vi "GetTerminal.vi"(5 "UseGObject":bool, 6 "TerminalIndex":i32, 7 "Other Refnum":refnum<vi>, 8 "error in (no error)":errorcluster, 9 "TerminalType":string, 10 "Label":string, 11 "vi reference":refnum<vi>) -> (0 "error out":errorcluster, 1 "Terminal desc":string, 2 "Terminal out":refnum<vi>, 3 "dup VI Refnum":refnum<vi>)   [LabVIEW 2020]
uses:
  <vilib>/Utility/traverseref.llb/TRef TravTarget.ctl
  <vilib>/Utility/traverseref.llb/VI Scripting - Traverse.lvlib
panel:
  out "Array 2":string[](array[string])
  out "Array":string[](array[string])
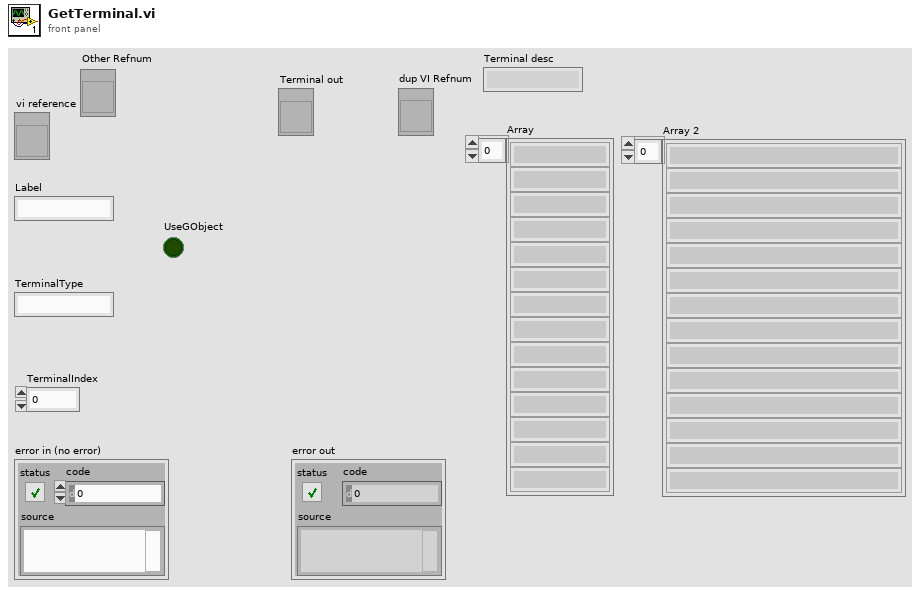
[diagram p1: front panel]
types:
  T1 = typedef "TRef TravTarget.ctl" = enum16{"FP", "BD", "Other"}
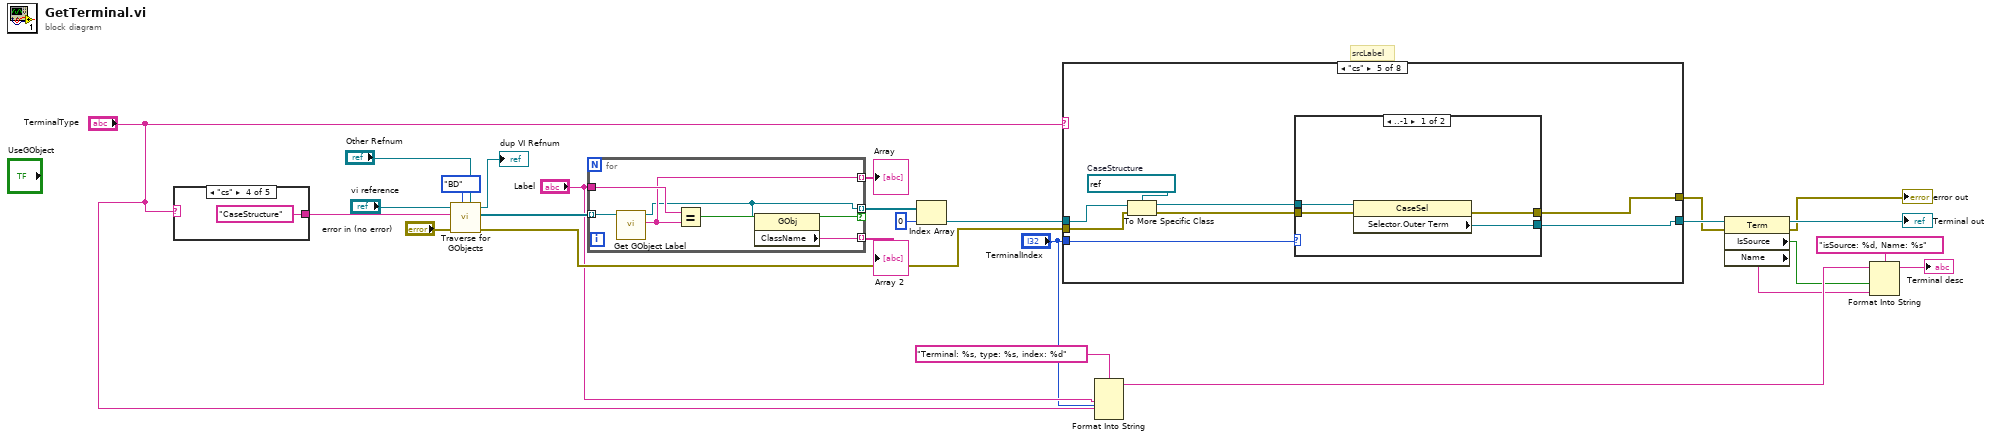
[diagram p0: block diagram]
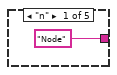
[diagram p2: hidden frame]
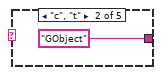
[diagram p3: hidden frame]
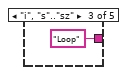
[diagram p4: hidden frame]
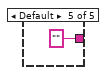
[diagram p5: hidden frame]
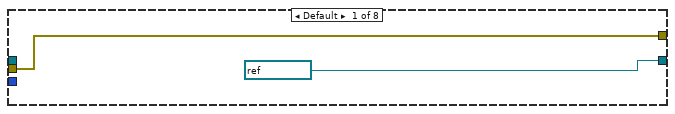
[diagram p6: hidden frame]
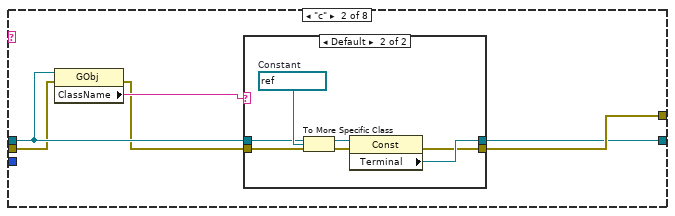
[diagram p7: hidden frame]
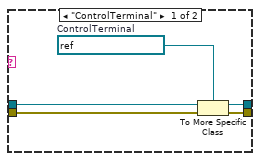
[diagram p8: hidden frame]
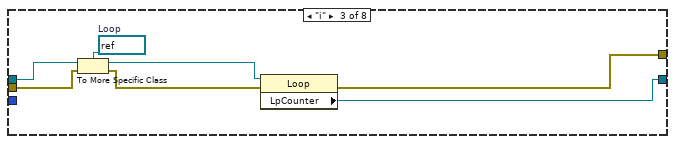
[diagram p9: hidden frame]
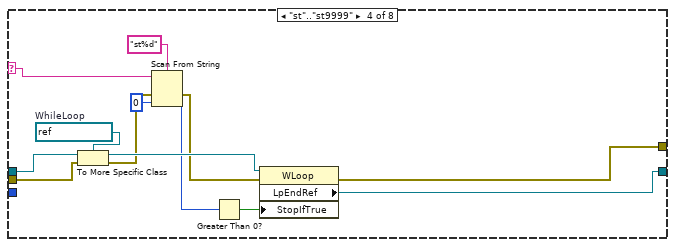
[diagram p10: hidden frame]
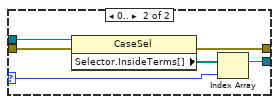
[diagram p11: hidden frame]
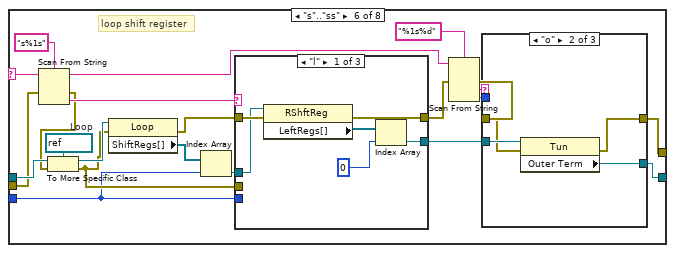
[diagram p12: hidden frame]
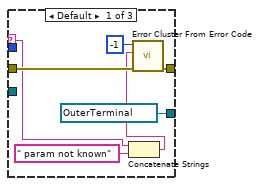
[diagram p13: hidden frame]
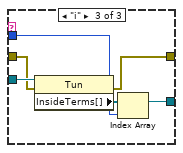
[diagram p14: hidden frame]
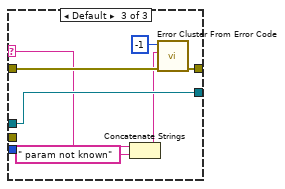
[diagram p16: hidden frame]
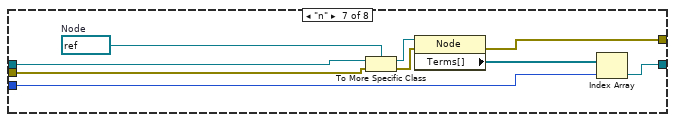
[diagram p17: hidden frame]
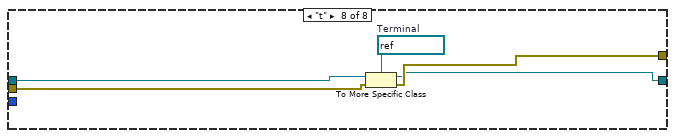
[diagram p18: hidden frame]
diagram:
  # "srcLabel"
  n1 = case shown="\"cs\"" "TerminalType" {
    tunnel: ["Node" "GObject" "Loop" "CaseStructure" ""] -> w25
    frame "n" {
    }
    frame "c", "t" {
    }
    frame "i", "s".."sz" {
    }
    frame "cs" {
    }
    frame Default {
    }
  }
  n2 = call <vilib>:"Traverse for GObjects.vi"("Other Refnum"="Other Refnum", "Traverse Target"=TRef_TravTarget."BD", "error in (no error)"="error in (no error)", "Class Name"=w25, "VI Refnum"="vi reference") -> ("error out"=w19:errorcluster, "References"=w26:refnum<vi>[], "dup VI Refnum"=→"dup VI Refnum":refnum<vi>)  [unwired: 3 in, 1 out]
  n3 = for {
    tunnel: w26 -> [w37] mode=indexing
    tunnel: "Label" -> [w35]
    tunnel: [w33] -> w23 mode=indexing if=w36
    tunnel: [w34] -> w17 mode=indexing
    tunnel: [w32] -> w16 mode=indexing
    n4 = call <vilib>:"Get GObject Label.vi"("GObject"=w37) -> ("Object Label"=w34:string, "dup GObject"=w33:refnum<vi>)  [unwired: 6 in, 3 out]
    n5 = Equal?(x=w35, y=w34) -> (x = y?=w36:bool)
    n6 = property class="GObj"(reference=w33) -> ("ClassName"=w32:string)  [unwired: 1 in, 2 out]
  }
  "Array" <- w17
  "Array 2" <- w16
  n7 = Index Array(array=w23, index=0) -> (element=w21:refnum<vi>)
  n8 = case shown="\"cs\"" "TerminalType" {
    selector: "TerminalType" -> [_ _ _ w70 _ w113 _ _]
    tunnel: w21 -> [_ w43 w64 w77 w85 w117 w158 w163]
    tunnel: [refnum<vi> refnum ("Terminal") w44 w63 w76 w79 w102 w155 w159] -> w13
    tunnel: "TerminalIndex" -> [_ _ _ _ w78 w109 w153 _]
    tunnel: w19 -> [w38 w42 w59 w72 w82 w105 w152 w161]
    tunnel: [w38 w45 w62 w75 w84 w98 w150 w160] -> w11
    frame Default {
    }
    frame "c" {
      n9 = property class="GObj"(reference=w43, error in=w42) -> (error out=w40:errorcluster, "ClassName"=w41:string)  [unwired: 1 out]
      n10 = case shown="Default" w41 {
        tunnel: [w49 w51] -> w45
        tunnel: [w48 w52] -> w44
        tunnel: w43 -> [w47 w56]
        tunnel: w40 -> [w46 w55]
        frame "ControlTerminal" {
          w50 = refnum<vi> refnum  # ControlTerminal
          n11 = To More Specific Class(target class=w50, reference=w47, error in=w46) -> (specific class reference=w48:refnum<vi>, error out=w49:errorcluster)
        }
        frame Default {
          w57 = refnum<vi> refnum  # Constant
          n12 = To More Specific Class(target class=w57, reference=w56, error in=w55) -> (specific class reference=w54:refnum<vi>, error out=w53:errorcluster)
          n13 = property class="Const"(reference=w54, error in=w53) -> (error out=w51:errorcluster, "Terminal"=w52:refnum<vi>)  [unwired: 1 out]
        }
      }
    }
    frame "i" {
      w61 = refnum<vi> refnum  # Loop
      n14 = To More Specific Class(target class=w61, reference=w64, error in=w59) -> (specific class reference=w60:refnum<vi>, error out=w58:errorcluster)
      n15 = property class="Loop"(reference=w60, error in=w58) -> (error out=w62:errorcluster, "LpCounter"=w63:refnum<vi>)  [unwired: 1 out]
    }
    frame "st".."st9999" {
      w74 = refnum<vi> refnum  # WhileLoop
      n16 = To More Specific Class(target class=w74, reference=w77, error in=w72) -> (specific class reference=w73:refnum<vi>, error out=w67:errorcluster)
      n17 = Scan From String(format string="st%d", input string=w70, error in=w67, default 1=0 ("default value 1")) -> (error out=w66:errorcluster, output 1=w69:i32)  [unwired: 1 in, 2 out]
      n18 = Greater Than 0?(x=w69) -> (x > 0?=w68:bool)
      n19 = property class="WLoop"(reference=w73, error in=w66, "StopIfTrue"=w68) -> (error out=w75:errorcluster, "LpEndRef"=w76:refnum<vi>)  [unwired: 1 out]
    }
    frame "cs" {
      w83 = refnum<vi> refnum  # CaseStructure
      n20 = To More Specific Class(target class=w83, reference=w85, error in=w82) -> (specific class reference=w81:refnum<vi>, error out=w80:errorcluster)
      n21 = case shown="..-1" w78 {
        selector: w78 -> [_ w90]
        tunnel: [w89 w95] -> w84
        tunnel: w81 -> [w88 w94]
        tunnel: w80 -> [w87 w93]
        tunnel: [w86 w91] -> w79
        frame ..-1 {
          n22 = property class="CaseSel"(reference=w88, error in=w87) -> (error out=w89:errorcluster, "Selector.Outer Term"=w86:refnum<vi>)  [unwired: 1 out]
        }
        frame 0.. {
          n23 = property class="CaseSel"(reference=w94, error in=w93) -> (error out=w95:errorcluster, "Selector.InsideTerms[]"=w92:refnum<vi>[])  [unwired: 1 out]
          n24 = Index Array(array=w92, index=w90) -> (element=w91:refnum<vi>)
        }
      }
    }
    frame "s".."ss" {
      w116 = refnum<vi> refnum  # Loop
      # "loop shift register"
      n25 = Scan From String(format string="s%1s", input string=w113, error in=w105) -> (remaining string=w96:string, error out=w104:errorcluster, output 1=w111:string)  [unwired: 2 in, 1 out]
      n26 = To More Specific Class(target class=w116, reference=w117, error in=w104) -> (specific class reference=w115:refnum<vi>, error out=w114:errorcluster)
      n27 = property class="Loop"(reference=w115, error in=w114) -> (error out=w110:errorcluster, "ShiftRegs[]"=w108:refnum<vi>[])  [unwired: 1 out]
      n28 = Index Array(array=w108, index=w109) -> (element=w107:refnum<vi>)
      n29 = case shown="\"l\"" w111 {
        selector: w111 -> [_ _ w145]
        tunnel: w114 -> [_ w141 _]
        tunnel: [w140 w141 w148] -> w103
        tunnel: w110 -> [w139 _ w147]
        tunnel: w109 -> [_ _ _]
        tunnel: [w138 w142 w149] -> w106
        tunnel: w107 -> [w137 w142 w149]
        frame "l" {
          n30 = property class="RShftReg"(reference=w137, error in=w139) -> (error out=w140:errorcluster, "LeftRegs[]"=w136:refnum<vi>[])  [unwired: 1 out]
          n31 = Index Array(array=w136, index=0) -> (element=w138:refnum<vi>)
        }
        frame "r" {
        }
        frame Default {
          n32 = Concatenate Strings(w145, " param not known" ("string")) -> (w144:string)
          n33 = call <vilib>:"Error Cluster From Error Code.vi"("error in (no error)"=w147, "error message (\"\")"=w144, "error code (0)"=-1) -> ("error out"=w148:errorcluster)  [unwired: 6 in]
        }
      }
      n34 = Scan From String(format string="%1s%d", input string=w96, error in=w103) -> (error out=w99:errorcluster, output 1=w100:string, output 2=w97:i32)  [unwired: 3 in, 2 out]
      n35 = case shown="\"o\"" w100 {
        selector: w100 -> [w121 _ _]
        tunnel: w106 -> [_ w128 w134]
        tunnel: [refnum<vi> refnum ("Outer Term") w127 w132] -> w102
        tunnel: w99 -> [w124 w126 w130]
        tunnel: [w123 w125 w129] -> w98
        tunnel: w97 -> [_ _ w131]
        frame Default {
          n36 = Concatenate Strings(w121, " param not known" ("string")) -> (w120:string)
          n37 = call <vilib>:"Error Cluster From Error Code.vi"("error in (no error)"=w124, "error message (\"\")"=w120, "error code (0)"=-1) -> ("error out"=w123:errorcluster)  [unwired: 6 in]
        }
        frame "o" {
          n38 = property class="Tun"(reference=w128, error in=w126) -> (error out=w125:errorcluster, "Outer Term"=w127:refnum<vi>)  [unwired: 1 out]
        }
        frame "i" {
          n39 = property class="Tun"(reference=w134, error in=w130) -> (error out=w129:errorcluster, "InsideTerms[]"=w133:refnum<vi>[])  [unwired: 1 out]
          n40 = Index Array(array=w133, index=w131) -> (element=w132:refnum<vi>)
        }
      }
    }
    frame "n" {
      w157 = refnum<vi> refnum  # Node
      n41 = To More Specific Class(target class=w157, reference=w158, error in=w152) -> (specific class reference=w156:refnum<vi>, error out=w151:errorcluster)
      n42 = property class="Node"(reference=w156, error in=w151) -> (error out=w150:errorcluster, "Terms[]"=w154:refnum<vi>[])  [unwired: 1 out]
      n43 = Index Array(array=w154, index=w153) -> (element=w155:refnum<vi>)
    }
    frame "t" {
      w162 = refnum<vi> refnum  # Terminal
      n44 = To More Specific Class(target class=w162, reference=w163, error in=w161) -> (specific class reference=w159:refnum<vi>, error out=w160:errorcluster)
    }
  }
  n45 = Format Into String(format string="Terminal: %s, type: %s, index: %d", "Label", "TerminalType", "TerminalIndex") -> (resulting string=w6:string)  [unwired: 2 in, 1 out]
  n46 = property class="Term"(reference=w13, error in=w11) -> (reference out=→"Terminal out":refnum<vi>, error out=→"error out":errorcluster, "IsSource"=w4:bool, "Name"=w3:string)
  n47 = Format Into String(format string="isSource: %d, Name: %s", initial string=w6, w4, w3) -> (resulting string=→"Terminal desc":string)  [unwired: 1 in, 1 out]
